vi "Send File.vi"(8 "Error In":errorcluster, 9 "Filename":string, 10 "Host Base Path":path, 11 "TargetItem":refnum<vi>) -> (0 "Error Out":errorcluster, 2 "Target File":path)   [LabVIEW 2023]
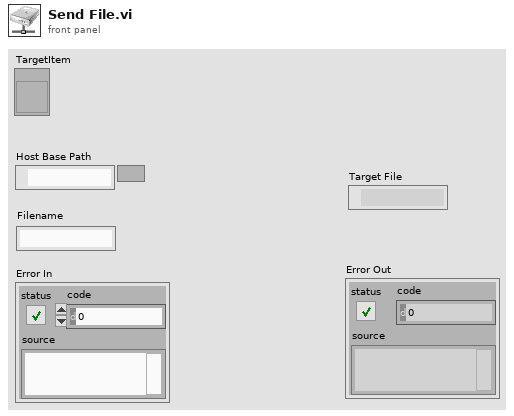
[diagram p1: front panel]
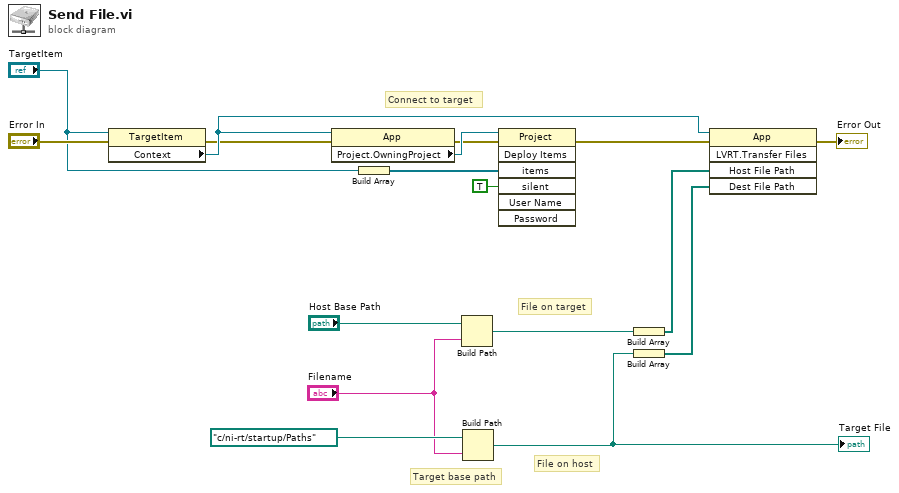
[diagram p0: block diagram]
diagram:
  # "Connect to target"
  # "File on target"
  # "Target base path"
  # "File on host"
  n1 = property class="TargetItem"(reference="TargetItem", error in="Error In") -> (error out=w5:errorcluster, "Context"=w8:refnum<vi>)  [unwired: 1 out]
  n2 = property class="App"(reference=w8, error in=w5) -> (error out=w4:errorcluster, "Project.OwningProject"=w7:refnum<vi>)  [unwired: 1 out]
  n3 = Build Array("TargetItem") -> (w3:refnum<vi>[])
  n4 = Build Path(base path="Host Base Path", name or relative path="Filename") -> (appended path=w15:path)
  n5 = Build Path(base path=path "c:/ni-rt/startup/Paths" ("Target Base Path"), name or relative path="Filename") -> (appended path=w14:path)
  "Target File" <- w14
  n6 = invoke class="Project" method="Deploy Items"(reference=w7, error in=w4, "items"=w3, "silent"=TRUE ("Silent")) -> (error out=w6:errorcluster)  [unwired: 3 in, 6 out]
  n7 = Build Array(w15) -> (w17:path[])
  n8 = Build Array(w14) -> (w16:path[])
  n9 = invoke class="App" method="LVRT.Transfer Files"(reference=w8, error in=w6, "Host File Path"=w17, "Dest File Path"=w16) -> (error out=→"Error Out":errorcluster)  [unwired: 1 in, 4 out]
